vi "Update Example Control Descriptions.vi"() -> ()   [LabVIEW 2016]
uses:
  <vilib>/Utility/traverseref.llb/TRef TravTarget.ctl
  <vilib>/Utility/traverseref.llb/VI Scripting - Traverse.lvlib
panel:
  in  "Update Top-Level Cluster Descriptions?":bool
  in  "Example Directory Path":path=path "../Examples"
  # "Set to True for example code,\nFalse for source code"
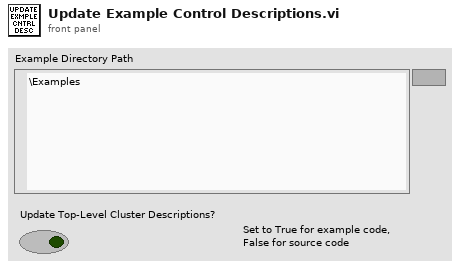
[diagram p1: front panel]
types:
  T1 = typedef "TRef TravTarget.ctl" = enum16{"FP", "BD", "Other"}
  T2 = enum32{"not a typedef", "typedef", "strict typedef", "class private data"}
  T3 = cluster{"Label.Text":string, refnum<vi>, "Desc":string}
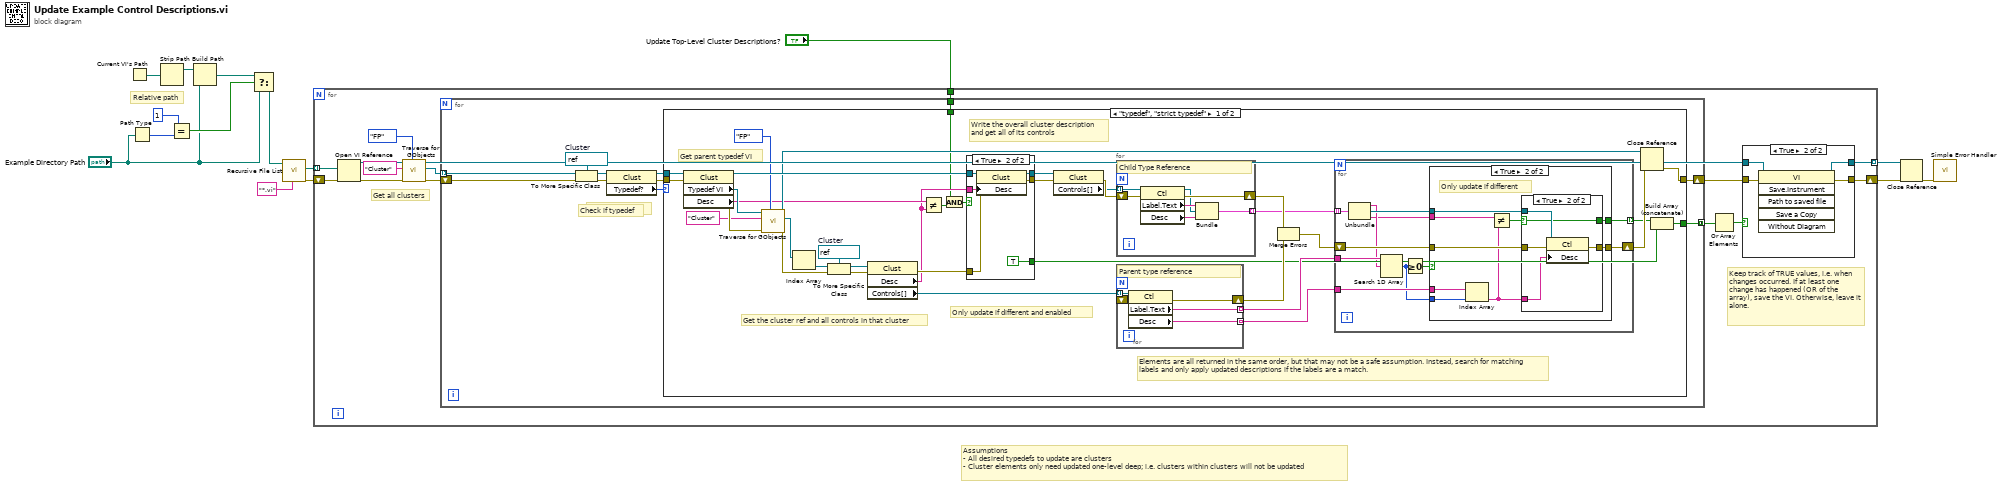
[diagram p0: block diagram]
diagram:
  # "Assumptions\n- All desired typedefs to update are clusters\n- Cluster elements only need updated one-level deep; i.e. clusters within clusters will not be updated"
  # "Relative path"
  n1 = Current VI's Path() -> (path=w10:path)
  n2 = Path Type(1:"Example Directory Path") -> (0:w9:i16)
  n3 = Strip Path(path=w10) -> (stripped path=w7:path)  [unwired: 1 out]
  n4 = Equal?(x=i16 1 ("y"), y=w9) -> (x = y?=w5:bool)
  n5 = Build Path(base path=w7, name or relative path="Example Directory Path") -> (appended path=w6:path)
  n6 = Select(t=w6, s=w5, f="Example Directory Path") -> (s? t:f=w3:path)
  n7 = call <vilib>:"Recursive File List.vi"("pattern"="*.vi", "Folder Path"=w3) -> ("error out"=w14:errorcluster, "All Files in Dir"=w12:path[])  [unwired: 5 in, 3 out]
  n8 = for {
    tunnel: w12 -> [w24] mode=indexing
    shift-right: [w18] -> w11
    shift-left: w14 -> [w28]
    tunnel: [w19] -> w2 mode=indexing
    tunnel: "Update Top-Level Cluster Descriptions?" -> [w15]
    # "Keep track of TRUE values, i.e. when changes occurred. If at least one change has happened (OR of the array), save the VI. Otherwise, leave it alone."
    # "Get all clusters"
    n9 = Open VI Reference(vi path=w24, error in (no error)=w28) -> (vi reference=w22:refnum<vi>, error out=w26:errorcluster)  [unwired: 4 in]
    n10 = call <vilib>:"Traverse for GObjects.vi"("Traverse Target"=TRef_TravTarget."FP", "error in (no error)"=w26, "Class Name"="Cluster", "VI Refnum"=w22) -> ("error out"=w27:errorcluster, "References"=w23:refnum<vi>[])  [unwired: 4 in, 2 out]
    n11 = for {
      tunnel: w23 -> [w39] mode=indexing
      shift-right: [w42] -> w25
      shift-left: w27 -> [w44]
      tunnel: [w36] -> w17 mode=concatenating
      tunnel: w15 -> [w35]
      w37 = refnum<vi> refnum  # Cluster
      # "Check if typedef"
      # "Check if typedef"
      n12 = To More Specific Class(target class=w37, reference=w39, error in=w44) -> (specific class reference=w38:refnum<vi>, error out=w43:errorcluster)
      n13 = property class="Clust"(reference=w38, error in=w43) -> (reference out=w40:refnum<vi>, error out=w45:errorcluster, "Typedef?"=w41:T2)
      n14 = case shown="\"typedef\", \"strict typedef\"" w41 {
        tunnel: w40 -> [w70 _]
        tunnel: w45 -> [w81 w130]
        tunnel: [w80 w130] -> w42
        tunnel: [w47 _] -> w36
        tunnel: w35 -> [w48 _]
        frame "typedef", "strict typedef" {
          w63 = refnum<vi> refnum  # Cluster
          # "Only update if different and enabled"
          # "Elements are all returned in the same order, but that may not be a safe assumption. Instead, search for matching labels and only apply updated descriptions if the labels are a match."
          # "Write the overall cluster description and get all of its controls"
          # "Get the cluster ref and all controls in that cluster"
          # "Get parent typedef VI"
          n15 = property class="Clust"(reference=w70, error in=w81) -> (reference out=w68:refnum<vi>, error out=w79:errorcluster, "Typedef VI"=w69:refnum<vi>, "Desc"=w52:string)
          n16 = call <vilib>:"Traverse for GObjects.vi"("Traverse Target"=TRef_TravTarget."FP", "error in (no error)"=w79, "Class Name"="Cluster", "VI Refnum"=w69) -> ("error out"=w78:errorcluster, "References"=w71:refnum<vi>[], "dup VI Refnum"=w67:refnum<vi>)  [unwired: 4 in, 1 out]
          n17 = Index Array(array=w71) -> (element=w65:refnum<vi>)  [unwired: 1 in]
          n18 = To More Specific Class(target class=w63, reference=w65, error in=w78) -> (specific class reference=w64:refnum<vi>, error out=w77:errorcluster)
          n19 = property class="Clust"(reference=w64, error in=w77) -> (error out=w54:errorcluster, "Desc"=w51:string, "Controls[]"=w61:refnum<vi>[])  [unwired: 1 out]
          n20 = Not Equal?(x=w52, y=w51) -> (x != y?=w49:bool)
          n21 = And(x=w48, y=w49) -> (x .and. y?=w50:bool)
          n22 = case shown="True" w50 {
            tunnel: w68 -> [w83 w89]
            tunnel: [w83 w88] -> w55
            tunnel: w51 -> [_ w87]
            tunnel: w54 -> [w82 w86]
            tunnel: [w82 w85] -> w53
            tunnel: [_ TRUE] -> w46
            frame False {
            }
            frame True {
              n23 = property class="Clust"(reference=w89, error in=w86, "Desc"=w87) -> (reference out=w88:refnum<vi>, error out=w85:errorcluster)
            }
          }
          n24 = property class="Clust"(reference=w55, error in=w53) -> (error out=w76:errorcluster, "Controls[]"=w62:refnum<vi>[])  [unwired: 1 out]
          n25 = for {
            tunnel: w62 -> [w122] mode=indexing
            shift-right: [w123] -> w75
            shift-left: w76 -> [w124]
            tunnel: [w120] -> w59 mode=indexing
            # "Child Type Reference"
            n26 = property class="Ctl"(reference=w122, error in=w124) -> (reference out=w119:refnum<vi>, error out=w123:errorcluster, "Label.Text"=w121:string, "Desc"=w118:string)
            n27 = Bundle("Label.Text"=w121, w119, "Desc"=w118) -> (w120:T3)  [unwired: 1 in]
          }
          n28 = for {
            tunnel: w61 -> [w127] mode=indexing
            shift-right: [w128] -> w74
            shift-left: _ -> [w129]
            tunnel: [w126] -> w58 mode=indexing
            tunnel: [w125] -> w57 mode=indexing
            # "Parent type reference"
            n29 = property class="Ctl"(reference=w127, error in=w129) -> (error out=w128:errorcluster, "Label.Text"=w126:string, "Desc"=w125:string)  [unwired: 1 out]
          }
          n30 = Merge Errors(w75, w74) -> (w73:errorcluster)
          n31 = for {
            shift-right: [w100] -> w72
            shift-left: w73 -> [w99]
            tunnel: w59 -> [w97] mode=indexing
            tunnel: w58 -> [w95]
            tunnel: w57 -> [w93]
            tunnel: [w90] -> w56 mode=indexing
            n32 = Unbundle(w97) -> ("Label.Text"=w94:string, w96:refnum<vi>, "Desc"=w91:string)
            n33 = Search 1D Array(1D array=w95, element=w94) -> (index of element=w92:i32)  [unwired: 1 in]
            n34 = Greater Or Equal To 0?(x=w92) -> (x >= 0?=w98:bool)
            n35 = case shown="True" w98 {
              tunnel: [w101 w110] -> w100
              tunnel: w99 -> [w101 w109]
              tunnel: w96 -> [_ w108]
              tunnel: w93 -> [_ w107]
              tunnel: w92 -> [_ w106]
              tunnel: w91 -> [_ w105]
              tunnel: [_ w102] -> w90
              frame False {
              }
              frame True {
                # "Only update if different"
                n36 = Index Array(array=w107, index=w106) -> (element=w104:string)
                n37 = Not Equal?(x=w105, y=w104) -> (x != y?=w103:bool)
                n38 = case shown="True" w103 {
                  selector: w103 -> [w111 w113]
                  tunnel: [w112 w117] -> w110
                  tunnel: w109 -> [w112 w116]
                  tunnel: w108 -> [_ w115]
                  tunnel: w104 -> [_ w114]
                  tunnel: [w111 w113] -> w102
                  frame False {
                  }
                  frame True {
                    n39 = property class="Ctl"(reference=w115, error in=w116, "Desc"=w114) -> (error out=w117:errorcluster)  [unwired: 1 out]
                  }
                }
              }
            }
          }
          n40 = Close Reference(reference=w67, error in (no error)=w72) -> (error out=w80:errorcluster)
          n41 = Build Array (concatenate)(w56, w46) -> (w47:bool[])
        }
        frame Default {
        }
      }
    }
    n42 = Or Array Elements(Boolean array=w17) -> (logical OR=w16:bool)
    n43 = case shown="True" w16 {
      tunnel: w25 -> [w29 w34]
      tunnel: w22 -> [w30 w33]
      tunnel: [w30 w32] -> w19
      tunnel: [w29 w31] -> w18
      frame False {
      }
      frame True {
        n44 = invoke class="VI" method="Save.Instrument"(reference=w33, error in=w34) -> (reference out=w32:refnum<vi>, error out=w31:errorcluster)  [unwired: 4 in, 4 out]
      }
    }
  }
  n45 = Close Reference(reference=w2) -> ()  [unwired: 1 in, 1 out]
  n46 = call <vilib>:"Simple Error Handler.vi"("error in (no error)"=w11) -> ()  [unwired: 4 in, 5 out]
